vi "Multi-Signal Generator.vi"() -> ()   [LabVIEW 2026]
uses:
  Controls/Signal Type.ctl
  Controls/Signal Settings.ctl
panel:
  in  "Signal Settings":T1
  out "Signal Status":string
  out "Generated Signal":dbl[](graph)
  # "Sampling freq: Tells how many samples we generate per second.\nNumber of samples: Tells us the total number of samples we want to generate."
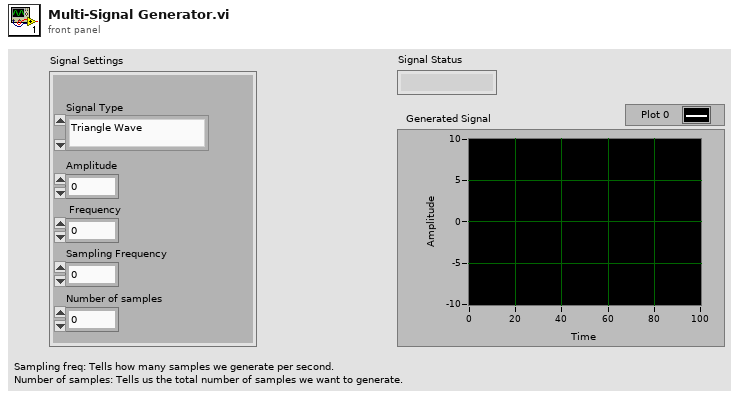
[diagram p1: front panel]
types:
  T1 = typedef "Signal Settings.ctl" = cluster{"Amplitude":dbl, " Frequency":dbl, "Sampling Frequency ":dbl, "Number of samples ":i32, "Signal Type":T2}
  T2 = typedef "Signal Type.ctl" = enum16{"Triangle Wave", "Square Wave", "Sine Wave"}
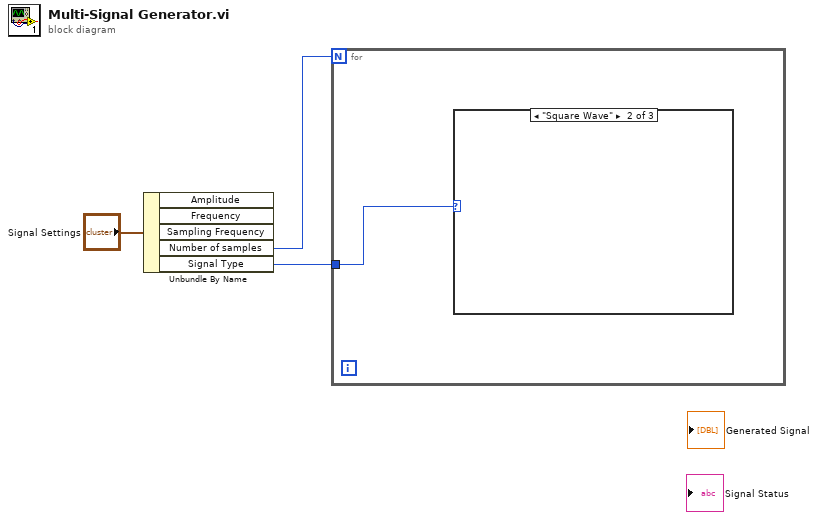
[diagram p0: block diagram]
diagram:
  n1 = Unbundle By Name("Signal Settings") -> ("Number of samples"=w2:i32, "Signal Type"=w1:T2)  [unwired: 3 out]
  n2 = for {
    N: w2 -> [_]
    tunnel: w1 -> [w4]
    n3 = case shown="\"Square Wave\"" w4 {
      frame "Triangle Wave", Default {
      }
      frame "Square Wave" {
      }
      frame "Sine Wave" {
      }
    }
  }
